vi "testSample.vi"() -> (3 "String":string="# Scope\nThis procedure is used to verify the Icon Editor properly launches from a fresh install with no saved settings.\n\nThis procedure was derived from the following NI tests:\n- 1692474: First launch IE Icon Editor\n\n# Setup\n**NOTE:** It is preferable to perform this test with a fresh LabVIEW install.\n\n1. Install the Icon Editor.\n2. Open Icon Editor Manual Tests.lvproj.\n3. Open and run Remove Icon Editor Settings.vi. This ensures there are no Icon Editor keys in the LabVIEW.ini file. All of the key names start with \"IconEditor.\"\n4. Close the VI and project.\n\n# Main\n1. Open a new VI from the Getting Started Window.\n2. From the Front Panel, double-click on the VI Icon.\n3. Verify the Icon Editor opens without seeing the loading dialog.\n4. Verify the Icon Editor is in the middle of the main monitor.\n5. Verify the Icon Text->Font combobox is properly populated based on fonts installed on the system.\n6. If Small Fonts is installed, verify Small Fonts is selected in the Font combobox. If not installed, verify \"LabVIEW Application\" is selected.\n7. Verify the font alignment is \"center\" and the font size is 9.\n8. Launch the Icon Editor Properties via the tools menu.\n9. Verify the Templates category is selected.\n10. Verify the following settings in the Templates category:\n- \"Save third-party icon templates?\" is unchecked.\n- \"Third-party template directory\" is set to \"\\<LabVIEW Data>\\\\Icon Templates\\\\3rd party\".\n11. Verify the following settings in the Layers category:\n- \"Merge all layers on commit\" is unchecked.\n12. Verify the following settings in the Text Tool category:\n- Font combobox is properly populated based on fonts installed on the system.\n- Font value is:\n    - If Small Fonts is installed, \"Small Fonts\"\n    - Else \"LabVIEW Application\"\n- Alignment is \"center\"\n- Size is 9\n13. Close the Icon Editor Properties dialog.\n14. Close the Icon Editor.\n15. From the VI Front Panel, double-click on the VI Icon.\n16. Verify the Icon Editor launched at least as fast as the first time opening it.\n**NOTE:** Because the Icon Editor is left in memory, it should load faster than the first run.\n\n# Cleanup\n1. Close the Icon Editor.\n2. Close the VI.")   [LabVIEW 2026]
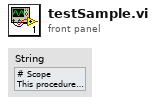
[diagram p1: front panel]
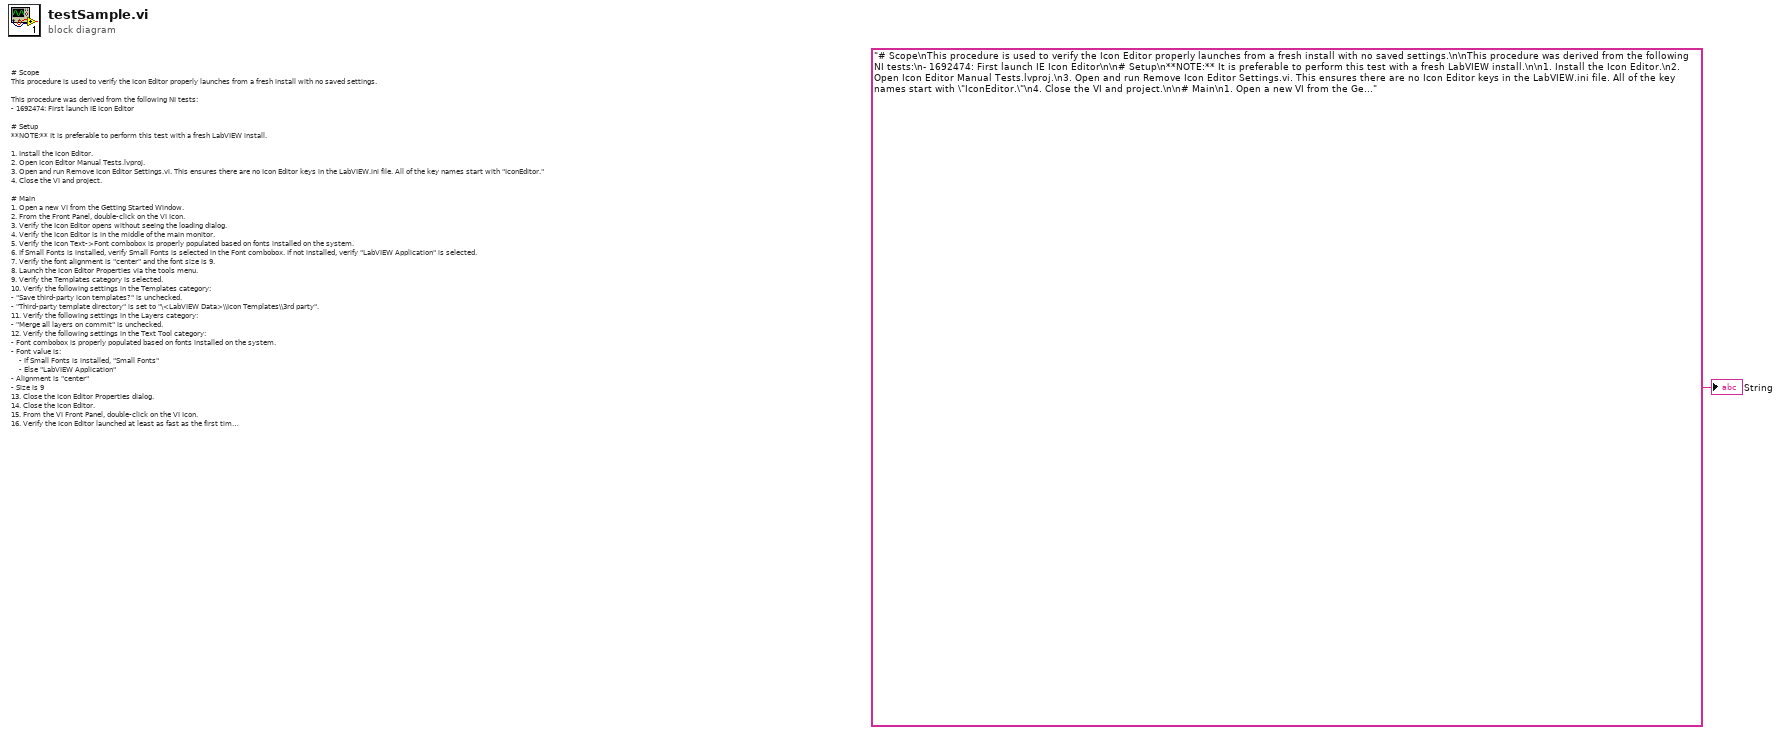
[diagram p0: block diagram]
diagram:
  # "# Scope\nThis procedure is used to verify the Icon Editor properly launches from a fresh install with no saved settings.\n\nThis procedure was derived from the following NI tests:\n- 1692474: First launch IE Icon Editor\n\n# Setup\n**NOTE:** It is preferable to perform this test with a fresh LabVIEW install.\n\n1. Install the Icon Editor.\n2. Open Icon Editor Manual Tests.lvproj.\n3. Open and run Remove Icon Editor Settings.vi. This ensures there are no Icon Editor keys in the LabVIEW.ini file. All of the key names start with \"IconEditor.\"\n4. Close the VI and project.\n\n# Main\n1. Open a new VI from the Getting Started Window.\n2. From the Front Panel, double-click on the VI Icon.\n3. Verify the Icon Editor opens without seeing the loading dialog.\n4. Verify the Icon Editor is in the middle of the main monitor.\n5. Verify the Icon Text->Font combobox is properly populated based on fonts installed on the system.\n6. If Small Fonts is installed, verify Small Fonts is selected in the Font combobox. If not installed, verify \"LabVIEW Application\" is selected.\n7. Verify the font alignment is \"center\" and the font size is 9.\n8. Launch the Icon Editor Properties via the tools menu.\n9. Verify the Templates category is selected.\n10. Verify the following settings in the Templates category:\n- \"Save third-party icon templates?\" is unchecked.\n- \"Third-party template directory\" is set to \"\\<LabVIEW Data>\\\\Icon Templates\\\\3rd party\".\n11. Verify the following settings in the Layers category:\n- \"Merge all layers on commit\" is unchecked.\n12. Verify the following settings in the Text Tool category:\n- Font combobox is properly populated based on fonts installed on the system.\n- Font value is:\n    - If Small Fonts is installed, \"Small Fonts\"\n    - Else \"LabVIEW Application\"\n- Alignment is \"center\"\n- Size is 9\n13. Close the Icon Editor Properties dialog.\n14. Close the Icon Editor.\n15. From the VI Front Panel, double-click on the VI Icon.\n16. Verify the Icon Editor launched at least as fast as the first time opening it.\n**NOTE:** Because the Icon Editor is left in memory, it should load faster than the first run.\n\n# Cleanup\n1. Close the Icon Editor.\n2. Close the VI."
  "String" <- "# Scope\nThis procedure is used to verify the Icon Editor properly launches from a fresh install with no saved settings.\n\nThis procedure was derived from the following NI tests:\n- 1692474: First launch IE Icon Editor\n\n# Setup\n**NOTE:** It is preferable to perform this test with a fresh LabVIEW install.\n\n1. Install the Icon Editor.\n2. Open Icon Editor Manual Tests.lvproj.\n3. Open and run Remove Icon Editor Settings.vi. This ensures there are no Icon Editor keys in the LabVIEW.ini file. All of the key names start with \"IconEditor.\"\n4. Close the VI and project.\n\n# Main\n1. Open a new VI from the Getting Started Window.\n2. From the Front Panel, double-click on the VI Icon.\n3. Verify the Icon Editor opens without seeing the loading dialog.\n4. Verify the Icon Editor is in the middle of the main monitor.\n5. Verify the Icon Text->Font combobox is properly populated based on fonts installed on the system.\n6. If Small Fonts is installed, verify Small Fonts is selected in the Font combobox. If not installed, verify \"LabVIEW Application\" is selected.\n7. Verify the font alignment is \"center\" and the font size is 9.\n8. Launch the Icon Editor Properties via the tools menu.\n9. Verify the Templates category is selected.\n10. Verify the following settings in the Templates category:\n- \"Save third-party icon templates?\" is unchecked.\n- \"Third-party template directory\" is set to \"\\<LabVIEW Data>\\\\Icon Templates\\\\3rd party\".\n11. Verify the following settings in the Layers category:\n- \"Merge all layers on commit\" is unchecked.\n12. Verify the following settings in the Text Tool category:\n- Font combobox is properly populated based on fonts installed on the system.\n- Font value is:\n    - If Small Fonts is installed, \"Small Fonts\"\n    - Else \"LabVIEW Application\"\n- Alignment is \"center\"\n- Size is 9\n13. Close the Icon Editor Properties dialog.\n14. Close the Icon Editor.\n15. From the VI Front Panel, double-click on the VI Icon.\n16. Verify the Icon Editor launched at least as fast as the first time opening it.\n**NOTE:** Because the Icon Editor is left in memory, it should load faster than the first run.\n\n# Cleanup\n1. Close the Icon Editor.\n2. Close the VI."
